vi "Stop server.vi"(8 "error in":errorcluster, 11 "connection ID":refnum<k5>) -> (0 "error out":errorcluster, 2 "Stop server message":string, 3 "connection ID out":refnum<k5>)   [LabVIEW 2020, in "LabVIEW-Python TCP Lib.lvlib"]
uses:
  LabVIEW-Python TCP Lib.lvlib
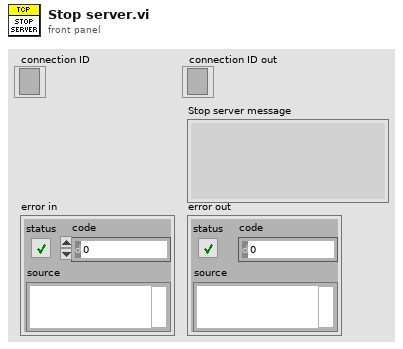
[diagram p1: front panel]
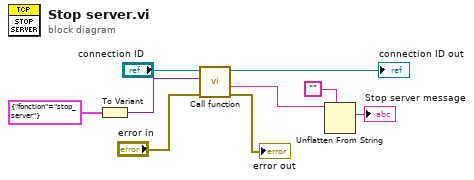
[diagram p0: block diagram]
diagram:
  n1 = To Variant(anything=cluster{"fonction":string} {"fonction"="stop_server"} ("Function cluster")) -> (Variant=w6:variant)
  n2 = call "Call function.vi"("error in"="error in", "variant in"=w6, "connection ID"="connection ID") -> ("error out"=→"error out":errorcluster, "data string out"=w5:string, "connection ID out"=→"connection ID out":refnum<k5>)  [unwired: 5 in, 1 out]
  n3 = Unflatten From String(type="", binary string=w5) -> (value=→"Stop server message":string)  [unwired: 3 in, 2 out]
